vi "PicoScope4000aSetupStreaming.vi"(0 "handle in":i16, 1 "enabled array":i16[](array[numeric]), 3 "Acquisition Settings":T2={"Auto Stop"=FALSE, "Desired Sample Interval"=4, "Pre-trigger Samples"=0, "Post-trigger Samples"=1000, "Down-Sample Ratio"=1, "Down-Sample Mode"=0, "Time Units"=2} {"Time Units" items=["Nanoseconds (ns)"=2, "Microseconds (us)"=3, "Milliseconds (ms)"=4, "Seconds (s)"=5]; "Down-Sample Mode" items=["None"=0, "Aggregate"=1, "Decimate"=2, "Average"=4]}, 4 "Buffer and Transfer Settings":T1={"startIndex"=0, "Samples"=1000000, "Down Sample Ratio"=1, "Down-Sample Mode"=0} {"Down-Sample Mode" items=["None"=0, "Aggregate"=1, "Decimate"=2, "Average"=4]; "Down Sample Ratio" step=1; "Samples" format="%_6p"}, 5 "error in":errorcluster, 10 "Pointers In":u64[][](array[numeric])) -> (11 "Pointer array":u64[][](array[numeric]), 14 "handle out":i16, 17 "Sample Interval":u32, 18 "sampleIntervalTimeUnits":u32, 19 "error out":errorcluster)   [LabVIEW 2010]
doc: "Set up the data buffers and calls RunStreaming to start the device streaming.\nData will be copied from the driver buffers into the corresponding application buffers using the wrapper dll."
uses:
  Program Files/Pico Technology/SDK/lib/ps4000a.dll
  ps4000aWrap.dll
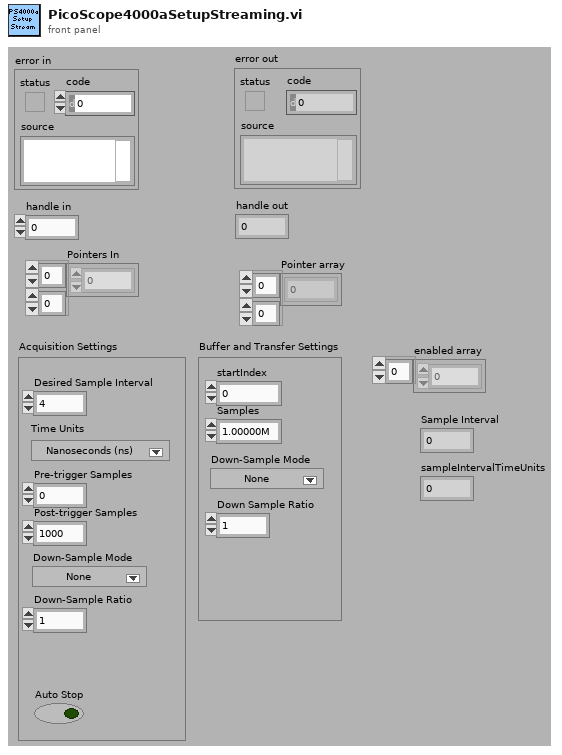
[diagram p1: front panel]
types:
  T1 = cluster{"startIndex":u64, "Samples":u64, "Down Sample Ratio":u64, "Down-Sample Mode":u32}
  T2 = cluster{"Auto Stop":bool, "Desired Sample Interval":u32, "Pre-trigger Samples":u32, "Post-trigger Samples":u32, "Down-Sample Ratio":u32, "Down-Sample Mode":i32, "Time Units":u32}
  T3 = cluster{"status":bool, "code":u32, "source":string}
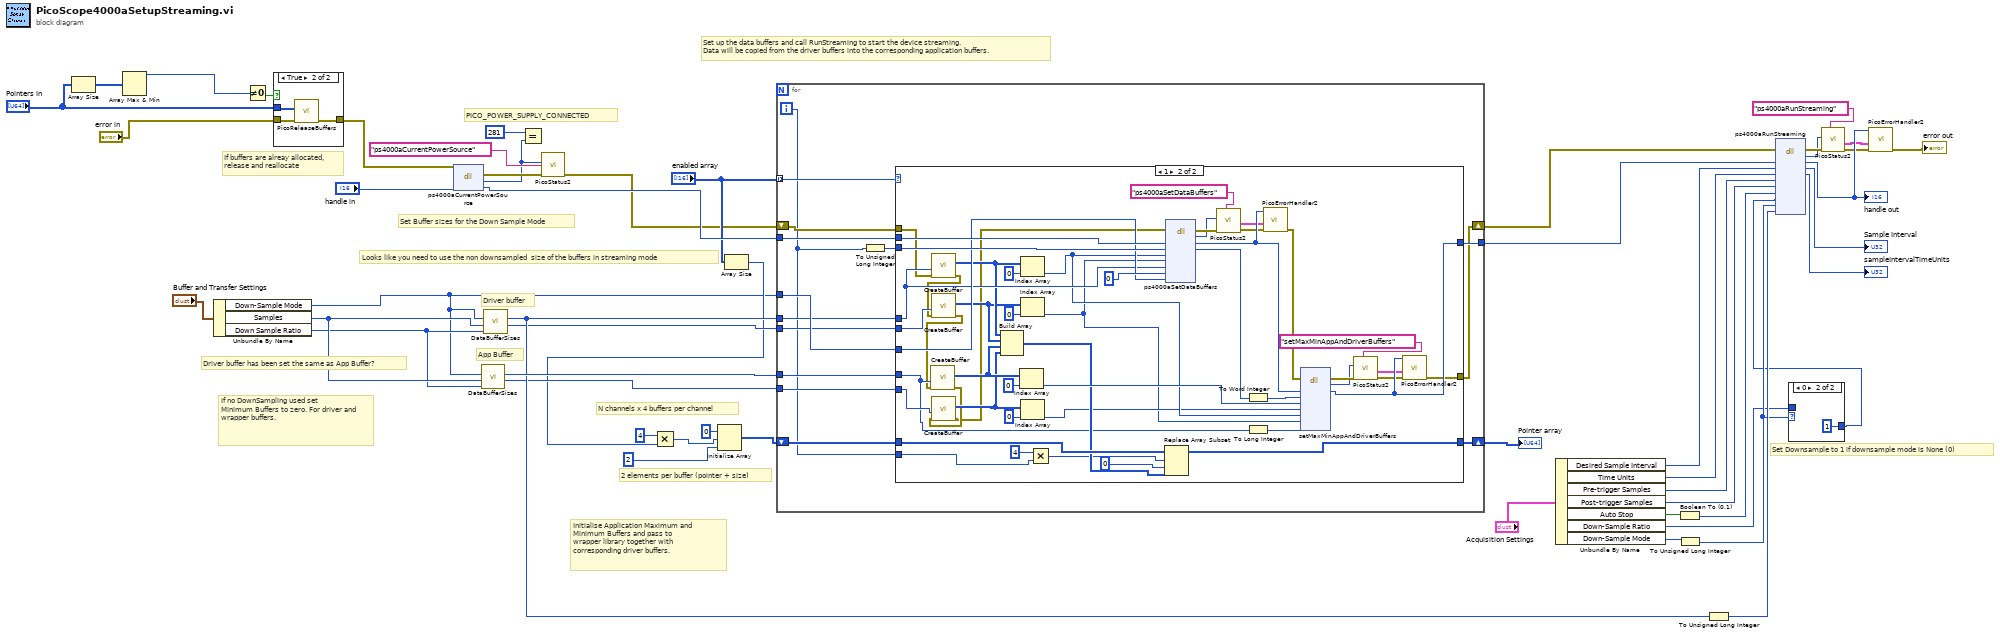
[diagram p0: block diagram]
diagram:
  # "Set Downsample to 1 if downsample mode is None (0)"
  # "Looks like you need to use the non downsampled  size of the buffers in streaming mode"
  # "If buffers are alreay allocated,\nrelease and reallocate"
  # "2 elements per buffer (pointer + size)"
  # "N channels x 4 buffers per channel"
  # "App Buffer"
  # "Driver buffer"
  # "Driver buffer has been set the same as App Buffer?"
  # "Set Buffer sizes for the Down Sample Mode"
  # "If no DownSampling used set \nMinimum Buffers to zero. For driver and wrapper buffers."
  # "PICO_POWER_SUPPLY_CONNECTED"
  # "Initialise Application Maximum and\nMinimum Buffers and pass to \nwrapper library together with corresponding driver buffers."
  # "Set up the data buffers and call RunStreaming to start the device streaming.\nData will be copied from the driver buffers into the corresponding application buffers."
  n1 = Array Size(array="Pointers In") -> (size(s)=w12:i32[])
  n2 = Array Max & Min(array=w12) -> (max value=w11:i32)  [unwired: 3 out]
  n3 = Unbundle By Name("Buffer and Transfer Settings") -> ("Down-Sample Mode"=w9:u32, "Samples"=w35:u64, "Down Sample Ratio"=w34:u64)
  n4 = Not Equal To 0?(x=w11) -> (x != 0?=w19:bool)
  n5 = case shown="True" w19 {
    tunnel: "Pointers In" -> [_ w54]
    tunnel: "error in" -> [w53 w55]
    tunnel: [w53 w56] -> w16
    frame False {
    }
    frame True {
      n6 = call "PicoReleaseBuffers.vi"("error in (no error)"=w55, "Pointer array"=w54) -> ("error out"=w56:errorcluster)  [unwired: 8 in, 1 out]
    }
  }
  n7 = dll-call lib="/Program Files/Pico Technology/SDK/lib/ps4000A.dll" fn="ps4000aCurrentPowerSource"(error in=w16, "handle"="handle in") -> (error out=w41:errorcluster, "PICO_STATUS"=w39:u32, "handle"=w38:i16)  [unwired: 2 in, 1 out]
  n8 = call "DataBufferSizes.vi"("Down Sample Ratio"=w34, "Number of Samples"=w35, "Down-Sample Mode"=w9) -> ("min Buffer Size"=w30:i32, "Max Buffer Size"=w33:i32)  [unwired: 7 in]
  n9 = call "DataBufferSizes.vi"("Down Sample Ratio"=w34, "Number of Samples"=w35, "Down-Sample Mode"=w9) -> ("min Buffer Size"=w31:i32, "Max Buffer Size"=w32:i32)  [unwired: 7 in]
  n10 = Equal?(x=u32 281, y=w39) -> ()  [unwired: 1 out]
  n11 = call "PicoStatus2.vi"("PICO source"="ps4000aCurrentPowerSource" ("source"), "Error in"=w41, "PICO STATUS"=w39) -> ("error out"=w15:errorcluster)  [unwired: 5 in, 1 out]
  n12 = Array Size(array="enabled array") -> (size(s)=w23:i32)
  n13 = Multiply(x=4, y=w23) -> (x*y=w24:i32)
  n14 = Initialize Array(u64 0 ("element"), w24, 2 ("dimension size")) -> (w13:u64[][])
  n15 = for {
    tunnel: "enabled array" -> [w62] mode=indexing
    tunnel: w38 -> [w70]
    tunnel: w9 -> [w69]
    tunnel: w33 -> [w68]
    tunnel: w32 -> [w67]
    tunnel: w31 -> [w66]
    tunnel: w30 -> [w65]
    tunnel: [w63] -> w26
    shift-right: [w61] -> w20
    shift-left: w15 -> [w60]
    shift-right: [w64] -> w29
    shift-left: w13 -> [w59]
    i -> [w57]
    n16 = To Unsigned Long Integer(number=w57) -> (unsigned 32bit integer=w58:u32)
    n17 = case shown="1" w62 {
      tunnel: w70 -> [w72 w122]
      tunnel: w60 -> [w71 w90]
      tunnel: w58 -> [_ w118]
      tunnel: w68 -> [_ w93]
      tunnel: w67 -> [_ w110]
      tunnel: w66 -> [_ w113]
      tunnel: w65 -> [_ w112]
      tunnel: w69 -> [_ w111]
      tunnel: w59 -> [w73 w104]
      tunnel: [w73 w103] -> w64
      tunnel: w57 -> [_ w100]
      tunnel: [w72 w85] -> w63
      tunnel: [w71 w84] -> w61
      frame 0, Default {
      }
      frame 1 {
        n18 = call "CreateBuffer.vi"("error in (no error)"=w90, "Buffer size"=w110) -> ("error out"=w89:errorcluster, "Pointer and BufferSize"=w108:u64[])  [unwired: 8 in]
        n19 = call "CreateBuffer.vi"("error in (no error)"=w89, "Buffer size"=w113) -> ("error out"=w88:errorcluster, "Pointer and BufferSize"=w107:u64[])  [unwired: 8 in]
        n20 = call "CreateBuffer.vi"("error in (no error)"=w88, "Buffer size"=w93) -> ("error out"=w87:errorcluster, "Pointer and BufferSize"=w106:u64[])  [unwired: 8 in]
        n21 = call "CreateBuffer.vi"("error in (no error)"=w87, "Buffer size"=w112) -> ("error out"=w86:errorcluster, "Pointer and BufferSize"=w105:u64[])  [unwired: 8 in]
        n22 = Build Array(w108, w107, w106, w105) -> (w99:u64[][])
        n23 = Index Array(array=w106, index=0) -> (element=w109:u64)
        n24 = Index Array(array=w108, index=0) -> (element=w102:u64)
        n25 = Index Array(array=w107, index=0) -> (element=w91:u64)
        n26 = Index Array(array=w105, index=0) -> (element=w92:u64)
        n27 = Multiply(x=4, y=w100) -> (x*y=w98:i32)
        n28 = Replace Array Subset(array=w104, new element=w99, index (row)=w98, index (col)=0 ("disabled index (row)")) -> (w103:u64[][])
        n29 = dll-call lib="/Program Files/Pico Technology/SDK/lib/ps4000a.dll" fn="ps4000aSetDataBuffers" ("ps3000.dll:_ps3000_open_unit@0")(error in=w86, "handle"=w122, "channel"=w118, "bufferMax"=w102, "bufferMin"=w91, "bufferLth"=w110, "segmentIndex"=u32 0, "downSampleRatioMode"=w111) -> (error out=w82:errorcluster, "PICO_STATUS"=w76:u32, "handle"=w95:i16, "channel"=w119:u32)  [unwired: 7 in, 1 out]
        n30 = call "PicoStatus2.vi"("PICO source"="ps4000aSetDataBuffers" ("source"), "Error in"=w82, "PICO STATUS"=w76) -> ("error out"=w83:errorcluster, "PICO_STATUS out"=w77:T3)  [unwired: 5 in]
        n31 = To Word Integer(number=w119) -> (16bit integer=w120:i16)
        n32 = To Long Integer(number=w93) -> (32bit integer=w94:i32)
        n33 = call "PicoErrorHandler2.vi"("error in (no error)"=w83, "PICO_STATUS in"=w77, "handle In"=w95) -> ("error out"=w96:errorcluster)  [unwired: 8 in]
        n34 = dll-call lib="ps4000aWrap.dll" fn="setMaxMinAppAndDriverBuffers"(error in=w96, "handle"=w95, "channel"=w120, "appMaxBuffer"=w109, "appMinBuffer"=w92, "driverMaxBuffer"=w102, "driverMinBuffer"=w91, "bufferLength"=w94) -> (error out=w80:errorcluster, "PICO_STATUS"=w78:u32, "handle"=w85:i16)  [unwired: 8 in, 1 out]
        n35 = call "PicoStatus2.vi"("PICO source"="setMaxMinAppAndDriverBuffers" ("source"), "Error in"=w80, "PICO STATUS"=w78) -> ("error out"=w81:errorcluster, "PICO_STATUS out"=w79:T3)  [unwired: 5 in]
        n36 = call "PicoErrorHandler2.vi"("error in (no error)"=w81, "PICO_STATUS in"=w79, "handle In"=w85) -> ("error out"=w84:errorcluster)  [unwired: 8 in]
      }
    }
  }
  "Pointer array" <- w29
  n37 = Unbundle By Name("Acquisition Settings") -> ("Desired Sample Interval"=w49:u32, "Time Units"=w43:u32, "Pre-trigger Samples"=w48:u32, "Post-trigger Samples"=w47:u32, "Auto Stop"=w46:bool, "Down-Sample Ratio"=w7:u32, "Down-Sample Mode"=w44:i32)
  n38 = Boolean To (0,1)(Boolean=w46) -> (0, 1=w50:i16)
  n39 = To Unsigned Long Integer(number=w44) -> (unsigned 32bit integer=w8:u32)
  n40 = To Unsigned Long Integer(number=w32) -> (unsigned 32bit integer=w10:u32)
  n41 = case shown="0" w8 {
    tunnel: [w123 u32 1 ("Down-Sample Ratio")] -> w6
    tunnel: w7 -> [w123 _]
    frame Default {
    }
    frame 0 {
    }
  }
  n42 = dll-call lib="/Program Files/Pico Technology/SDK/lib/ps4000a.dll" fn="ps4000aRunStreaming" ("ps5000a.dll:_ps3000_open_unit@0")(error in=w20, "handle"=w26, "sampleInterval"=w49, "sampleIntervalTimeUnits"=w43, "maxPreTriggerSamples"=w48, "maxPostTriggerSamples"=w47, "autoStop"=w50, "downSampleRatio"=w6, "downSampleRatioMode"=w8, "overviewBufferSize"=w10) -> (error out=w5:errorcluster, "PICO_STATUS"=w4:u32, "handle"=w14:i16, "sampleInterval"=→"Sample Interval":u32, "sampleIntervalTimeUnits"=→"sampleIntervalTimeUnits":u32)  [unwired: 8 in, 1 out]
  "handle out" <- w14
  n43 = call "PicoStatus2.vi"("PICO source"="ps4000aRunStreaming" ("source"), "Error in"=w5, "PICO STATUS"=w4) -> ("error out"=w3:errorcluster, "PICO_STATUS out"=w1:T3)  [unwired: 5 in]
  n44 = call "PicoErrorHandler2.vi"("error in (no error)"=w3, "PICO_STATUS in"=w1, "handle In"=w14) -> ("error out"=→"error out":errorcluster)  [unwired: 8 in]
